vi "Day 4.vi"() -> ()   [LabVIEW 2021]
uses:
  <vilib>/Utility/file.llb/Read Delimited Spreadsheet (string).vi
panel:
  out "Boards":string[][][](array[string])
  out "Numbers":string[](array[string])
  out "Solution":i32
  out "Input":string[](array[string])
  in  "Input File":enum32{"example input", "input"}(radio)
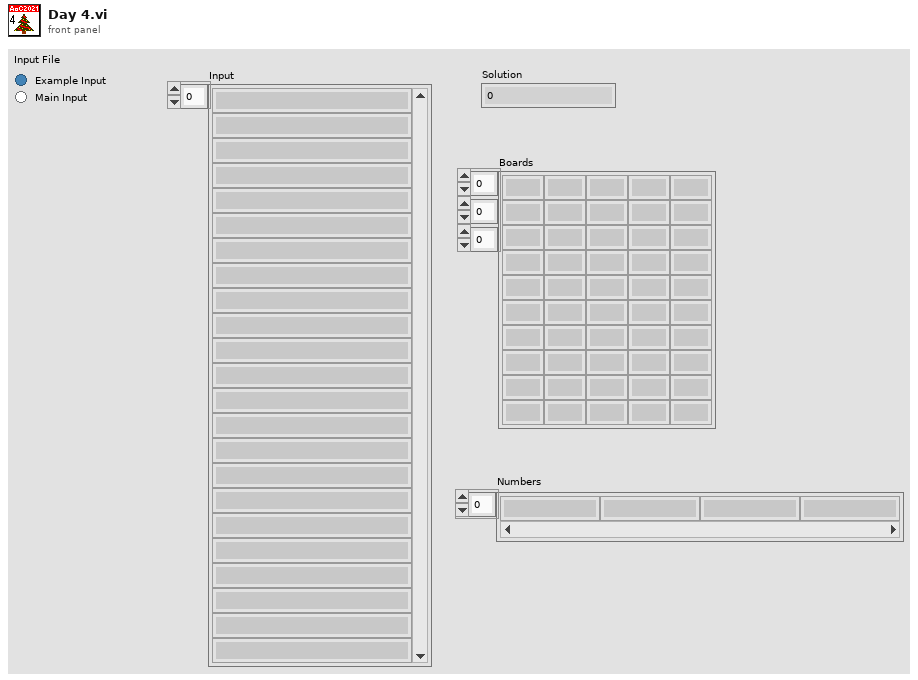
[diagram p1: front panel]
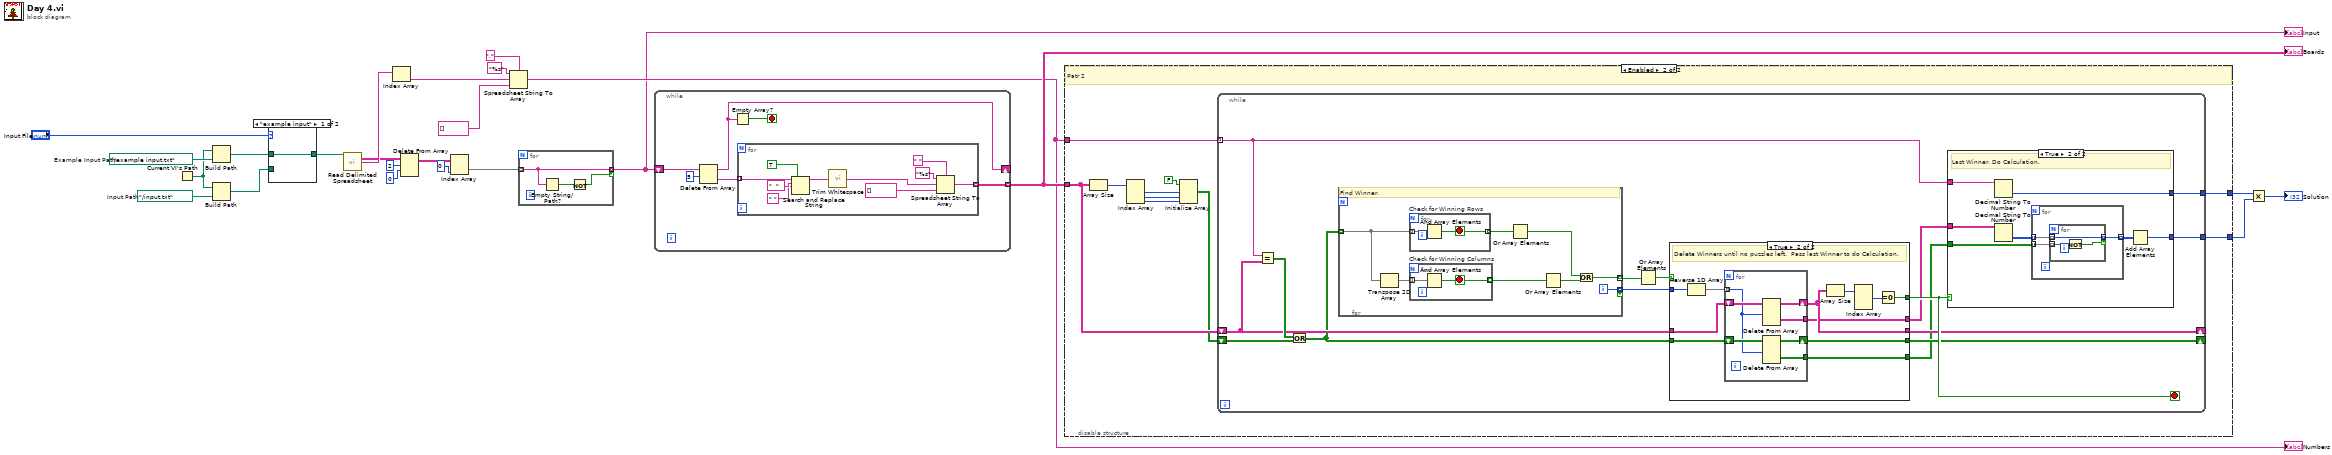
[diagram p0: block diagram]
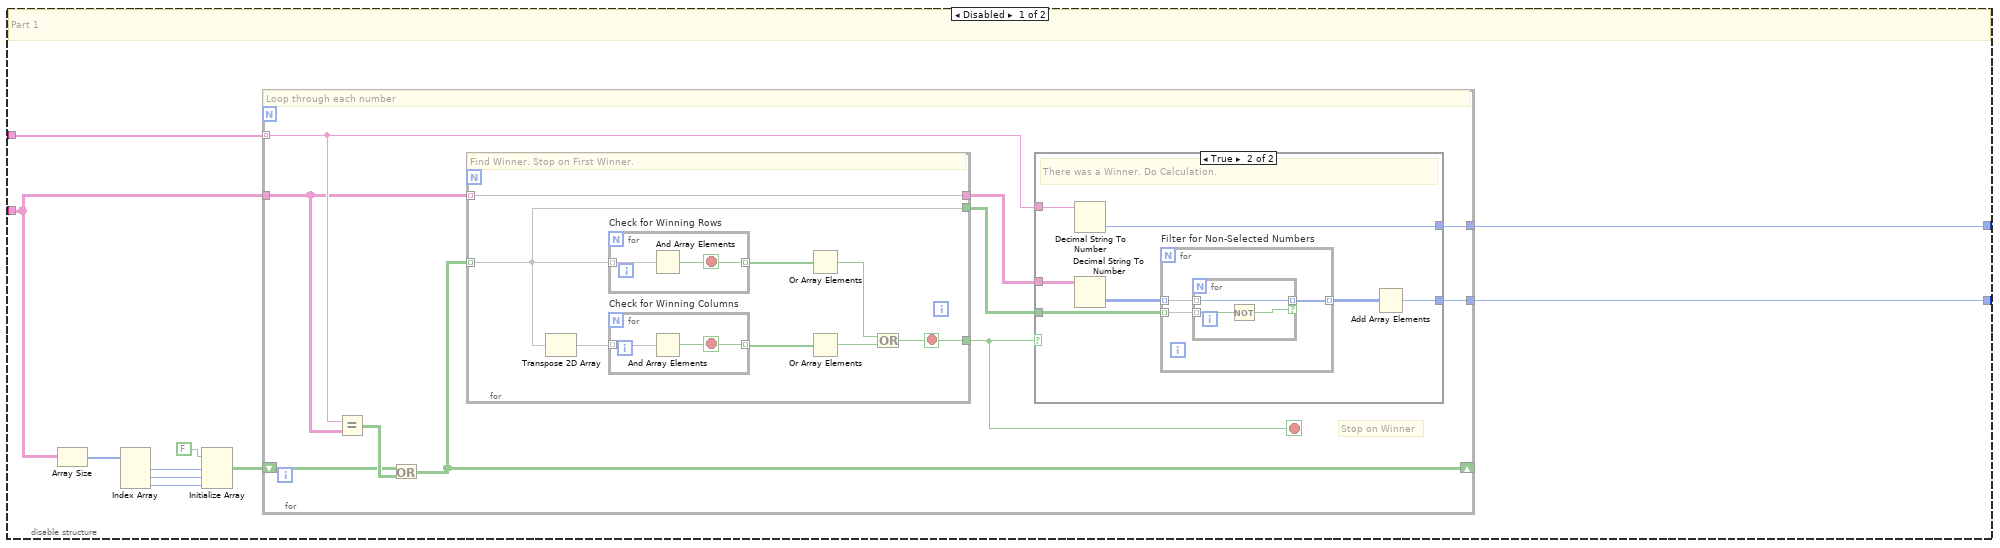
[diagram p2: hidden frame]
diagram:
  w23 = path "../example input.txt"  # Example Input Path
  w24 = path "../input.txt"  # Input Path
  n1 = Current VI's Path() -> (path=w18:path)
  n2 = Build Path(base path=w18, name or relative path=w23) -> (appended path=w20:path)
  n3 = Build Path(base path=w18, name or relative path=w24) -> (appended path=w21:path)
  n4 = case shown="\"example input\"" "Input File" {
    tunnel: w21 -> [_ w26]
    tunnel: w20 -> [w25 _]
    tunnel: [w25 w26] -> w19
    frame "example input" {
    }
    frame "input" {
    }
  }
  n5 = call-poly <vilib>:"Read Delimited Spreadsheet.vi"("file path (dialog if empty)"=w19) -> ("all rows"=w15:string[][], "first row"=w16:string[])  [unwired: 9 in, 4 out]
  n6 = Index Array(array=w16) -> (element=w13:string)  [unwired: 1 in]
  n7 = Delete From Array(array=w15, length=2, index (row)=0) -> (array with subset deleted=w6:string[][])  [unwired: 1 in, 1 out]
  n8 = Index Array(array=w6, index (col)=0 ("disabled index (col)")) -> (element=w5:string[])  [unwired: 1 in]
  n9 = Spreadsheet String To Array(delimiter (Tab)=",", format string="%s", spreadsheet string=w13, array type (2D Dbl)=string[] []) -> (array=w7:string[])
  "Numbers" <- w7
  n10 = for {
    tunnel: w5 -> [w29] mode=indexing
    tunnel: [w29] -> w4 mode=indexing if=w27
    n11 = Empty String/Path?(string/path=w29) -> (empty?=w28:bool)
    n12 = Not(x=w28) -> (.not. x?=w27:bool)
  }
  "Input" <- w4
  n13 = while {
    shift-right: [w32] -> _
    shift-left: w4 -> [w35]
    tunnel: [w30] -> w8 mode=indexing
    stop <- w31 stop-if-true
    n14 = Delete From Array(array=w35, length=5) -> (deleted portion=w33:string[], array with subset deleted=w32:string[])  [unwired: 1 in]
    n15 = Empty Array?(array=w32) -> (empty?=w31:bool)
    n16 = for {
      tunnel: w33 -> [w41] mode=indexing
      tunnel: [w42] -> w30 mode=indexing
      n17 = Search and Replace String(replace all?=TRUE ("replace all? (F)"), input string=w41, search string="  ", replace string=" ") -> (result string=w40:string)  [unwired: 4 in, 3 out]
      n18 = call <vilib>:"Trim Whitespace.vi"("string"=w40) -> ("trimmed string"=w36:string)  [unwired: 1 in]
      n19 = Spreadsheet String To Array(delimiter (Tab)=" ", format string="%s", spreadsheet string=w36, array type (2D Dbl)=string[] []) -> (array=w42:string[])
    }
  }
  "Boards" <- w8
  n20 = disable-structure shown="Enabled" {
    disable-tunnel: w8 -> [w52 w97]
    disable-tunnel: w7 -> [w55 w100]
    disable-tunnel: [w54 w99] -> w2
    disable-tunnel: [w53 w98] -> w1
    frame Disabled {
      # "Part 1"
      n21 = Array Size(array=w52) -> (size(s)=w51:i32[])
      n22 = Index Array(array=w51) -> (element #1=w50:i32, element #2=w48:i32, element #3=w47:i32)  [unwired: 3 in]
      n23 = Initialize Array(FALSE, w50, w48, w47) -> (w46:bool[][][])
      n24 = for {
        tunnel: w55 -> [w65] mode=indexing
        tunnel: [w63] -> w54
        tunnel: [w62] -> w53
        shift-right: [w56] -> _
        shift-left: w46 -> [w57]
        tunnel: w52 -> [w60]
        stop <- w58 stop-if-true
        # "Stop on Winner"
        # "Loop through each number"
        n25 = Equal?(x=w65, y=w60) -> (x = y?=w61:bool[][][])
        n26 = Or(x=w57, y=w61) -> (x .or. y?=w56:bool[][][])
        n27 = for {
          tunnel: w56 -> [w81] mode=indexing
          tunnel: [w79] -> w58
          tunnel: [w81] -> w64
          tunnel: w60 -> [w80] mode=indexing
          tunnel: [w80] -> w59
          stop <- w79 stop-if-true
          # "Find Winner. Stop on First Winner."
          n28 = Transpose 2D Array(2D array=w81) -> (transposed array=w86:bool[][])
          n29 = for "Check for Winning Rows" {
            tunnel: w81 -> [w90] mode=indexing
            tunnel: [w89] -> w85 mode=indexing
            stop <- w89 stop-if-true
            n30 = And Array Elements(Boolean array=w90) -> (logical AND=w89:bool)
          }
          n31 = for "Check for Winning Columns" {
            tunnel: w86 -> [w88] mode=indexing
            tunnel: [w87] -> w84 mode=indexing
            stop <- w87 stop-if-true
            n32 = And Array Elements(Boolean array=w88) -> (logical AND=w87:bool)
          }
          n33 = Or Array Elements(Boolean array=w85) -> (logical OR=w83:bool)
          n34 = Or Array Elements(Boolean array=w84) -> (logical OR=w82:bool)
          n35 = Or(x=w83, y=w82) -> (x .or. y?=w79:bool)
        }
        n36 = case shown="True" w58 {
          tunnel: w65 -> [_ w71]
          tunnel: w64 -> [_ w69]
          tunnel: w59 -> [_ w72]
          tunnel: [_ w67] -> w63
          tunnel: [_ w66] -> w62
          frame False {
          }
          frame True {
            # "There was a Winner. Do Calculation."
            n37 = Decimal String To Number(string=w71) -> (number=w66:i32)  [unwired: 2 in, 1 out]
            n38 = Decimal String To Number(string=w72) -> (number=w70:i32[][])  [unwired: 2 in, 1 out]
            n39 = for "Filter for Non-Selected Numbers" {
              tunnel: w70 -> [w75] mode=indexing
              tunnel: w69 -> [w74] mode=indexing
              tunnel: [w73] -> w68 mode=indexing
              n40 = for {
                tunnel: w75 -> [w78] mode=indexing
                tunnel: w74 -> [w77] mode=indexing
                tunnel: [w78] -> w73 mode=indexing if=w76
                n41 = Not(x=w77) -> (.not. x?=w76:bool)
              }
            }
            n42 = Add Array Elements(numeric array=w68) -> (sum=w67:i32)
          }
        }
      }
    }
    frame Enabled {
      # "Patr 2"
      n43 = Array Size(array=w97) -> (size(s)=w96:i32[])
      n44 = Index Array(array=w96) -> (element #1=w95:i32, element #2=w93:i32, element #3=w92:i32)  [unwired: 3 in]
      n45 = Initialize Array(FALSE, w95, w93, w92) -> (w91:bool[][][])
      n46 = while {
        tunnel: w100 -> [w115] mode=indexing
        tunnel: [w114] -> w99
        tunnel: [w113] -> w98
        shift-right: [w102] -> _
        shift-left: w91 -> [w112]
        shift-right: [w104] -> _
        shift-left: w97 -> [w109]
        stop <- w106 stop-if-true
        n47 = Equal?(x=w115, y=w109) -> (x = y?=w111:bool[][][])
        n48 = Or(x=w111, y=w112) -> (x .or. y?=w107:bool[][][])
        n49 = for {
          tunnel: w107 -> [w138] mode=indexing
          tunnel: [w136] -> w110 mode=indexing
          tunnel: [w137] -> w108 mode=indexing if=w136
          i -> [w137]
          # "Find Winner."
          n50 = Transpose 2D Array(2D array=w138) -> (transposed array=w143:bool[][])
          n51 = for "Check for Winning Rows" {
            tunnel: w138 -> [w147] mode=indexing
            tunnel: [w146] -> w142 mode=indexing
            stop <- w146 stop-if-true
            n52 = And Array Elements(Boolean array=w147) -> (logical AND=w146:bool)
          }
          n53 = for "Check for Winning Columns" {
            tunnel: w143 -> [w145] mode=indexing
            tunnel: [w144] -> w141 mode=indexing
            stop <- w144 stop-if-true
            n54 = And Array Elements(Boolean array=w145) -> (logical AND=w144:bool)
          }
          n55 = Or Array Elements(Boolean array=w142) -> (logical OR=w140:bool)
          n56 = Or Array Elements(Boolean array=w141) -> (logical OR=w139:bool)
          n57 = Or(x=w140, y=w139) -> (x .or. y?=w136:bool)
        }
        n58 = Or Array Elements(Boolean array=w110) -> (logical OR=w105:bool)
        n59 = case shown="True" w105 {
          tunnel: w109 -> [w116 w128]
          tunnel: w108 -> [_ w126]
          tunnel: [w116 w123] -> w104
          tunnel: w107 -> [w117 w127]
          tunnel: [w117 w125] -> w102
          tunnel: [_ w122] -> w106
          tunnel: [_ w120] -> w103
          tunnel: [_ w119] -> w101
          frame False {
            # "No Winners"
          }
          frame True {
            # "Delete Winners until no puzzles left.  Pass last Winner to do Calculation."
            n60 = Reverse 1D Array(array=w126) -> (reversed array=w121:i32[])
            n61 = for {
              tunnel: w121 -> [w133] mode=indexing
              shift-right: [w132] -> w125
              shift-left: w127 -> [w134]
              shift-right: [w131] -> w123
              shift-left: w128 -> [w135]
              tunnel: [w130] -> w120
              tunnel: [w129] -> w119
              n62 = Delete From Array(array=w135, index (dim 0)=w133) -> (deleted portion=w130:string[][], array with subset deleted=w131:string[][][])  [unwired: 3 in]
              n63 = Delete From Array(array=w134, index (dim 0)=w133) -> (deleted portion=w129:bool[][], array with subset deleted=w132:bool[][][])  [unwired: 3 in]
            }
            n64 = Array Size(array=w123) -> (size(s)=w124:i32[])
            n65 = Index Array(array=w124) -> (element #1=w118:i32)  [unwired: 3 in, 2 out]
            n66 = Equal To 0?(x=w118) -> (x = 0?=w122:bool)
          }
        }
        n67 = case shown="True" w106 {
          tunnel: w115 -> [_ w154]
          tunnel: w101 -> [_ w149]
          tunnel: w103 -> [_ w148]
          tunnel: [_ w151] -> w114
          tunnel: [_ w150] -> w113
          frame False {
          }
          frame True {
            # "Last Winner. Do Calculation."
            n68 = Decimal String To Number(string=w154) -> (number=w150:i32)  [unwired: 2 in, 1 out]
            n69 = Decimal String To Number(string=w148) -> (number=w153:i32[][])  [unwired: 2 in, 1 out]
            n70 = for {
              tunnel: w153 -> [w157] mode=indexing
              tunnel: w149 -> [w156] mode=indexing
              tunnel: [w155] -> w152 mode=indexing
              n71 = for {
                tunnel: w157 -> [w160] mode=indexing
                tunnel: w156 -> [w159] mode=indexing
                tunnel: [w160] -> w155 mode=indexing if=w158
                n72 = Not(x=w159) -> (.not. x?=w158:bool)
              }
            }
            n73 = Add Array Elements(numeric array=w152) -> (sum=w151:i32)
          }
        }
      }
    }
  }
  n74 = Multiply(x=w1, y=w2) -> (x*y=→"Solution":i32)
